vi "Decode Request.vi"(11 "二进制字符串":string) -> (3 "值":T1)   [LabVIEW 2020, in "TCP Communication.lvlib"]
uses:
  TCP Communication.lvlib
  Requset.ctl
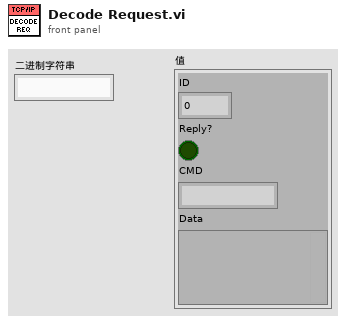
[diagram p1: front panel]
types:
  T1 = typedef "TCP Communication.lvlib/Requset.ctl" = cluster{"ID":i32, "Reply?":bool, "CMD":string, "Data":variant}
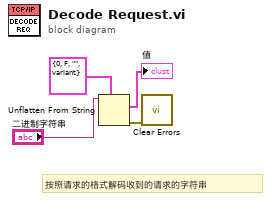
[diagram p0: block diagram]
diagram:
  # "按照请求的格式解码收到的请求的字符串"
  n1 = Unflatten From String(type=T1 {"ID"=0, "Reply?"=FALSE, "CMD"="", "Data"=variant} ("请求"), binary string="二进制字符串") -> (value=→"值":T1, error out=w1:errorcluster)  [unwired: 3 in, 1 out]
  n2 = call <vilib>:"Clear Errors.vi"("error in (no error)"=w1) -> ()  [unwired: 5 in, 2 out]
